vi "Set TP.vi"(8 "error in (no error)":errorcluster, 10 "Main":refnum<vi>) -> (0 "error out":errorcluster)   [LabVIEW 2025, in "Flow Grind.lvlib" / "Pressure Gain.lvclass"]
uses:
  Pressure Gain.lvclass
  <vilib>/Analysis/6fits.llb/Curve Fitting Criteria.ctl
  Pressure Gain.lvclass/Pressure Gain.ctl
  <vilib>/Analysis/NI_AALPro.lvlib
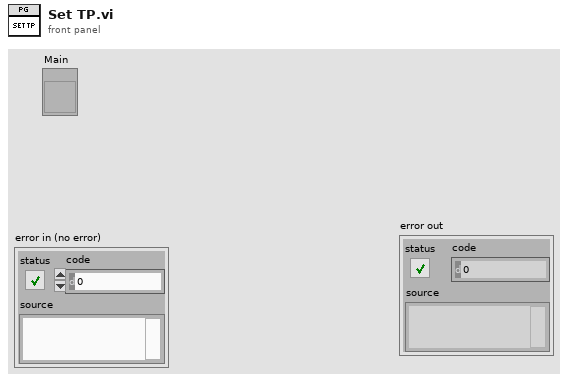
[diagram p1: front panel]
types:
  T1 = typedef "NI_AALPro.lvlib/Curve Fitting Criteria.ctl" = u16
  T2 = cluster{"Name":string, "Color":u32, "Style":u8, "Point Style":u8, "Name Visible":bool, "Allow Drag":bool, "Annotation Mode":u32, "Plot":i32, "Index":i32, "Position":cluster{"X":dbl, "Y":dbl}, "X Scale":u32, "Y Scale":u32, "Show Arrow":bool, "Lock Name":bool, "Plot Area":i32, "Label Offset":cluster{"X":dbl, "Y":dbl}}
  T3 = typedef "LVAnnotationListTypeDef.ctl" = cluster{"Name":string, "Color":u32, "Style":u8, "Point Style":u8, "Name Visible":bool, "Allow Drag":bool, "Annotation Mode":u32, "Plot":i32, "Index":i32, "Position":cluster{"X":dbl, "Y":dbl}, "X Scale":u32, "Y Scale":u32, "Show Arrow":bool, "Lock Name":bool, "Plot Area":i32, "Label Offset":cluster{"X":dbl, "Y":dbl}}[]
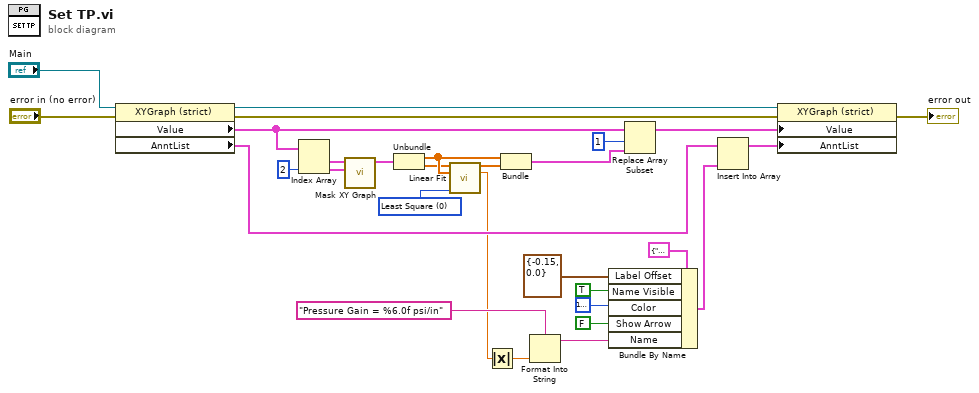
[diagram p0: block diagram]
diagram:
  w13 = T1 0 items=["Least Square", "Least Absolute Residual", "Bisquare"] ("method")
  n1 = property class="XYGraph (strict)"(reference="Main", error in="error in (no error)") -> (reference out=w28:refnum<vi>, error out=w27:errorcluster, "Value"=w10:cluster{dbl[], dbl[]}[], "AnntList"=w19:T3)
  n2 = Index Array(array=w10, index #2=2 ("index")) -> (element #1=w18:cluster{dbl[], dbl[]}, element #2=w17:cluster{dbl[], dbl[]})  [unwired: 1 in]
  n3 = call "Mask XY Graph.vi"("Mask"=w17, "Data"=w18) -> ("Masked Data"=w12:cluster{"X":dbl[], "Y":dbl[]})  [unwired: 7 in, 2 out]
  n4 = Unbundle(w12) -> ("X"=w16:dbl[], "Y"=w14:dbl[])
  n5 = call <vilib>:"Linear Fit.vi"("Y"=w14, "X"=w16, "method"=w13) -> ("Best Linear Fit"=w15:dbl[], "slope"=w5:dbl)  [unwired: 8 in, 3 out]
  n6 = Absolute Value(x=w5) -> (abs(x)=w4:dbl)
  n7 = Bundle("X"=w16, "Best Linear Fit"=w15) -> (w7:cluster{"X":dbl[], "Best Linear Fit":dbl[]})  [unwired: 1 in]
  n8 = Format Into String(format string="Pressure Gain = %6.0f psi/in", w4) -> (resulting string=w2:string)  [unwired: 2 in, 1 out]
  n9 = Bundle By Name(cluster=T2 {"Name"="", "Color"=0, "Style"=0, "Point Style"=0, "Name Visible"=FALSE, "Allow Drag"=FALSE, "Annotation Mode"=0, "Plot"=0, "Index"=0, "Position"={"X"=0.0, "Y"=0.0}, "X Scale"=0, "Y Scale"=0, "Show Arrow"=FALSE, "Lock Name"=FALSE, "Plot Area"=0, "Label Offset"={"X"=0.0, "Y"=0.0}}, "Label Offset"=cluster{"X":dbl, "Y":dbl} {"X"=-0.15, "Y"=0.0}, "Name Visible"=TRUE, "Color"=u32 16777224, "Show Arrow"=FALSE, "Name"=w2) -> (w29:T2)
  n10 = Replace Array Subset(array=w10, new element=w7, index=1) -> (w6:cluster{dbl[], dbl[]}[])
  n11 = Insert Into Array(array=w19, new element=w29) -> (w11:T3)  [unwired: 1 in]
  n12 = property class="XYGraph (strict)"(reference=w28, error in=w27, "Value"=w6, "AnntList"=w11) -> (error out=→"error out":errorcluster)  [unwired: 1 out]
